vi "Arr-string.vi"(11 "数组":string[](array[string])) -> (3 "结果字符串":string)   [LabVIEW 2018]
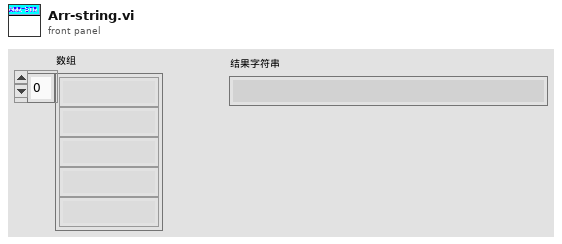
[diagram p1: front panel]
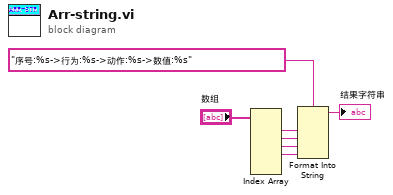
[diagram p0: block diagram]
diagram:
  n1 = Index Array(array="数组") -> (element #1=w5:string, element #2=w4:string, element #3=w3:string, element #4=w2:string)  [unwired: 6 in, 2 out]
  n2 = Format Into String(format string="序号:%s->行为:%s->动作:%s->数值:%s" ("格式字符串"), w5, w4, w3, w2) -> (resulting string=→"结果字符串":string)  [unwired: 2 in, 1 out]
